vi "Deploy History.vi"() -> ()   [LabVIEW 2023]
doc: "Tools >> Systemcore >> Deploy History: lists the robot's deploys (newest first) and redeploys the one the user picks, or checks it out into the project."
panel:
  out "Status":string
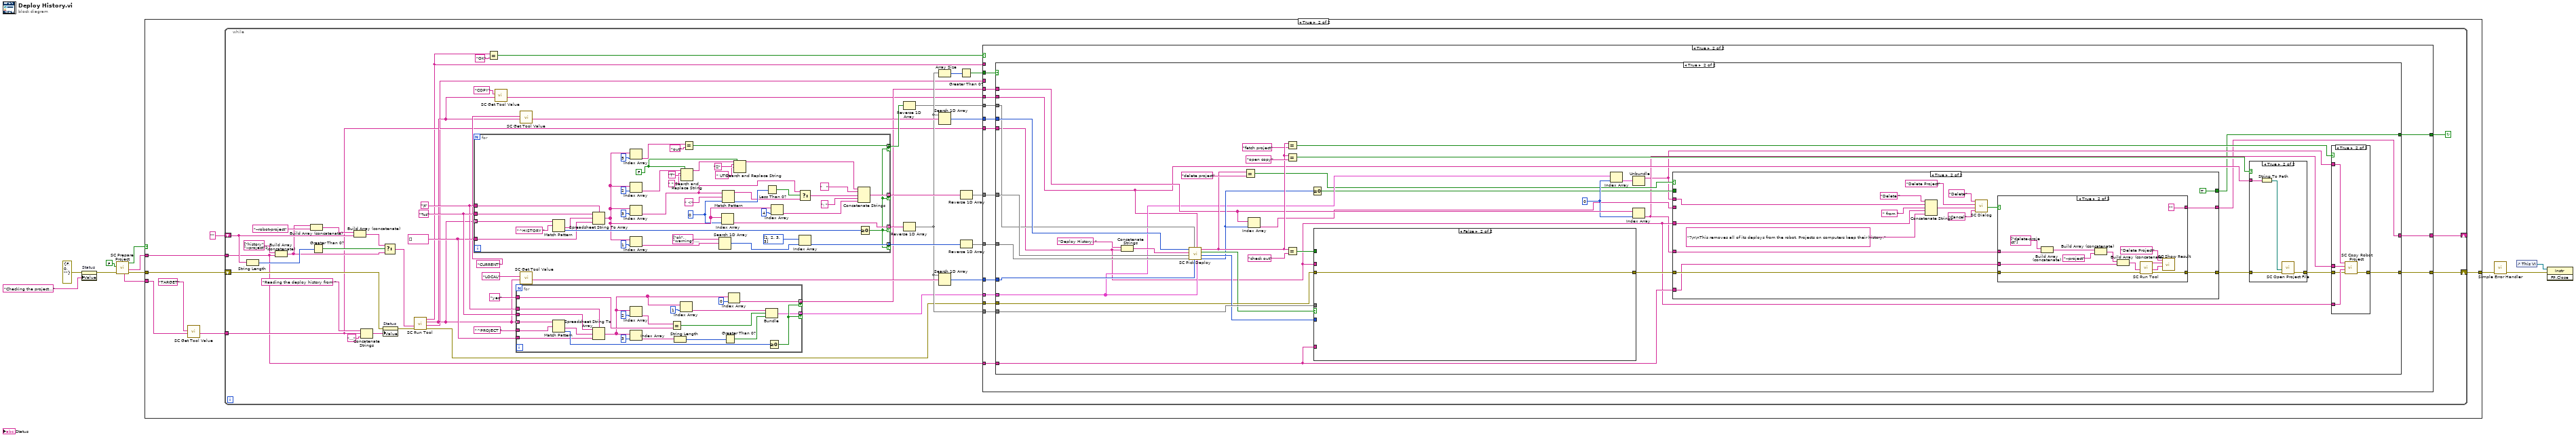
[diagram p0: block diagram]
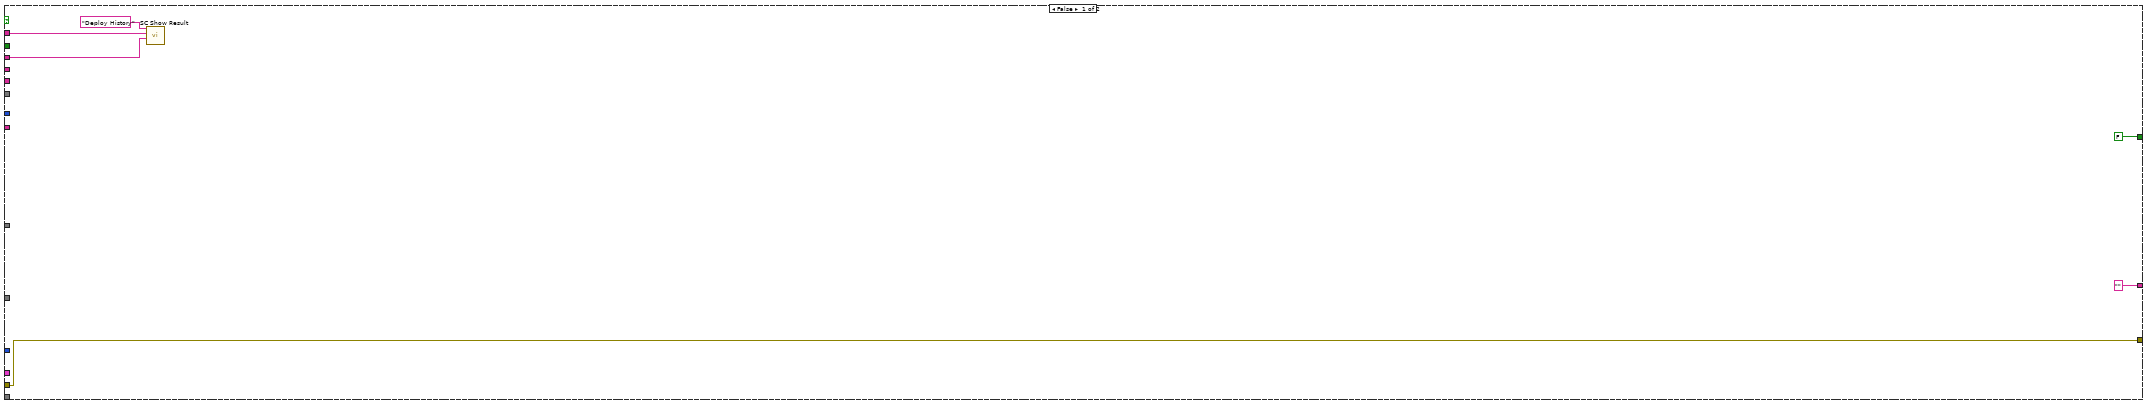
[diagram p3: hidden frame]
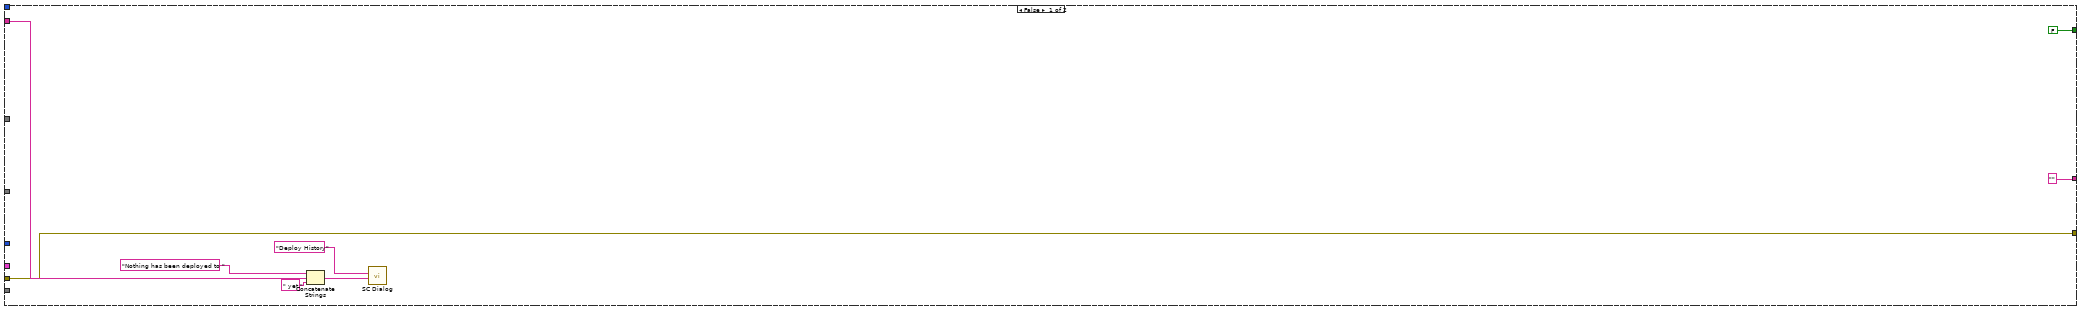
[diagram p4: hidden frame]
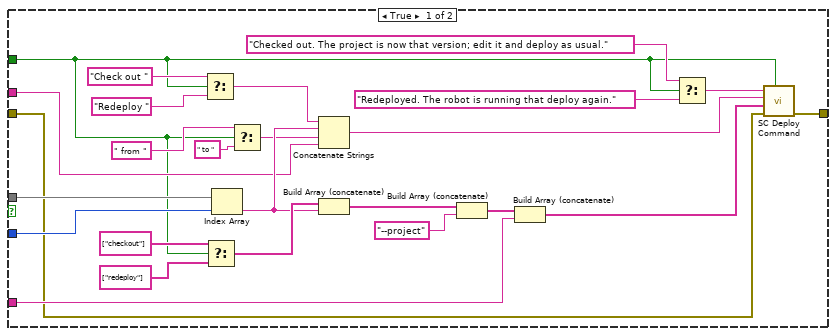
[diagram p9: hidden frame]
diagram:
  n1 = property on="Status" class="Str"(error in=errorcluster {"status"=FALSE, "code"=0, "source"=""}, "Value"="Checking the project...") -> (error out=w8:errorcluster)  [unwired: 1 in, 1 out]
  n2 = call "SC Prepare Project.vi"("error in (no error)"=w8, "save VIs?"=FALSE) -> ("error out"=w5:errorcluster, "project root"=w7:string, "ready?"=w4:bool, "tool lines"=w6:string[])  [unwired: 5 in, 1 out]
  n3 = case shown="True" w4 {
    tunnel: w7 -> [_ w17]
    tunnel: w6 -> [_ w19]
    tunnel: w5 -> [w12 w15]
    tunnel: [w12 w13] -> w3
    frame False {
    }
    frame True {
      n4 = call "SC Get Tool Value.vi"("tool lines"=w19, "key"="TARGET") -> ("value"=w16:string)  [unwired: 8 in, 1 out]
      n5 = while {
        tunnel: w17 -> [w34]
        tunnel: w16 -> [w35]
        shift-right: [w21] -> w13
        shift-left: w15 -> [w56]
        shift-right: [w22] -> _
        shift-left: "" -> [w67]
        stop <- w23 continue-if-true
        w50 = "\t"
        w51 = string[] []
        w52 = "%s"
        n6 = String Length(string=w67) -> (length=w66:i32)
        n7 = Build Array (concatenate)(string[] ["history", "--project"], w34) -> (w59:string[])
        n8 = Build Array (concatenate)(w59, "--robot-project") -> (w68:string[])
        n9 = Greater Than 0?(x=w66) -> (x > 0?=w65:bool)
        n10 = Build Array (concatenate)(w68, w67) -> (w64:string[])
        n11 = Concatenate Strings("Reading the deploy history from ", w35, "...") -> (w55:string)
        n12 = property on="Status" class="Str"(error in=w56, "Value"=w55) -> (error out=w53:errorcluster)  [unwired: 1 in, 1 out]
        n13 = Select(t=w64, s=w65, f=w59) -> (s? t:f=w54:string[])
        n14 = call "SC Run Tool.vi"("error in (no error)"=w53, "arguments"=w54) -> ("error out"=w33:errorcluster, "output"=w32:string, "tool lines"=w45:string[], "result"=w31:string)  [unwired: 4 in, 2 out]
        n15 = for {
          tunnel: w45 -> [w250] mode=indexing
          tunnel: w52 -> [w247]
          tunnel: w51 -> [w245]
          tunnel: w50 -> [w244]
          tunnel: [w213] -> w42 mode=indexing if=w210
          tunnel: [w212] -> w41 mode=indexing if=w210
          tunnel: [w211] -> w49 mode=indexing if=w210
          tunnel: [w209] -> w48 mode=indexing if=w210
          w229 = FALSE
          w227 = 0
          n16 = Match Pattern(string=w250, regular expression="^HISTORY ") -> (after substring=w246:string, offset past match=w248:i32)  [unwired: 1 in, 2 out]
          n17 = Spreadsheet String To Array(delimiter (Tab)=w244, format string=w247, spreadsheet string=w246, array type (2D Dbl)=w245) -> (array=w239:string[])
          n18 = Index Array(array=w239, index=5) -> (element=w237:string)
          n19 = Index Array(array=w239, index=2) -> (element=w235:string)
          n20 = Index Array(array=w239, index=3) -> (element=w224:string)
          n21 = Index Array(array=w239, index=1) -> (element=w216:string)
          n22 = Search and Replace String(replace all?=w229, input string=w235, search string="T", replace string=" ") -> (result string=w232:string)  [unwired: 4 in, 3 out]
          n23 = Equal?(x=w237, y="out") -> (x = y?=w209:bool)
          n24 = Search 1D Array(1D array=string[] ["ok", "warning", "broken", "error"], element=w216) -> (index of element=w214:i32)  [unwired: 1 in]
          n25 = Index Array(array=w239, index=w227) -> (element=w213:string)
          n26 = Match Pattern(string=w224, regular expression=" <", offset (0)=w227) -> (before substring=w223:string, offset past match=w226:i32)  [unwired: 2 out]
          n27 = Search and Replace String(replace all?=w229, input string=w232, search string="Z", replace string=" UTC") -> (result string=w222:string)  [unwired: 4 in, 3 out]
          n28 = Less Than 0?(x=w226) -> (x < 0?=w225:bool)
          n29 = Index Array(array=w239, index=4) -> (element=w218:string)
          n30 = Select(t=w224, s=w225, f=w223) -> (s? t:f=w220:string)
          n31 = Index Array(array=i32[] [1, 2, 3, 3], index=w214) -> (element=w211:i32)
          n32 = Concatenate Strings(w222, "   ", w220, ": ", w218) -> (w212:string)
          n33 = Greater Or Equal To 0?(x=w248) -> (x >= 0?=w210:bool)
        }
        n34 = Equal?(x=w31, y="OK") -> (x = y?=w20:bool)
        n35 = call "SC Get Tool Value.vi"("tool lines"=w45, "key"="COPY") -> ("value"=w24:string)  [unwired: 8 in, 1 out]
        n36 = for {
          tunnel: w45 -> [w272] mode=indexing
          tunnel: w52 -> [w269]
          tunnel: w51 -> [w267]
          tunnel: w50 -> [w266]
          tunnel: "^PROJECT " -> [w271]
          tunnel: "yes" -> [w261]
          tunnel: [w253] -> w26 mode=indexing if=w252
          tunnel: [w251] -> w25 mode=indexing if=w252
          n37 = Match Pattern(string=w272, regular expression=w271) -> (after substring=w268:string, offset past match=w270:i32)  [unwired: 1 in, 2 out]
          n38 = Spreadsheet String To Array(delimiter (Tab)=w266, format string=w269, spreadsheet string=w268, array type (2D Dbl)=w267) -> (array=w260:string[])
          n39 = Index Array(array=w260, index=2) -> (element=w262:string)
          n40 = Index Array(array=w260, index=3) -> (element=w258:string)
          n41 = Equal?(x=w262, y=w261) -> (x = y?=w255:bool)
          n42 = String Length(string=w258) -> (length=w257:i32)
          n43 = Index Array(array=w260, index=1) -> (element=w256:string)
          n44 = Greater Than 0?(x=w257) -> (x > 0?=w254:bool)
          n45 = Index Array(array=w260, index=0) -> (element=w253:string)
          n46 = Bundle("String"=w256, w255, w254) -> (w251:cluster{"String":string, bool, bool})  [unwired: 1 in]
          n47 = Greater Or Equal To 0?(x=w270) -> (x >= 0?=w252:bool)
        }
        n48 = call "SC Get Tool Value.vi"("tool lines"=w45, "key"="CURRENT") -> ("value"=w46:string)  [unwired: 8 in, 1 out]
        n49 = call "SC Get Tool Value.vi"("tool lines"=w45, "key"="LOCAL") -> ("value"=w43:string)  [unwired: 8 in, 1 out]
        n50 = Reverse 1D Array(array=w48) -> (reversed array=w28:bool[])
        n51 = Reverse 1D Array(array=w42) -> (reversed array=w37:string[])
        n52 = Array Size(array=w37) -> (size(s)=w40:i32)
        n53 = Search 1D Array(1D array=w37, element=w46) -> (index of element=w29:i32)  [unwired: 1 in]
        n54 = Search 1D Array(1D array=w37, element=w43) -> (index of element=w27:i32)  [unwired: 1 in]
        n55 = Greater Than 0?(x=w40) -> (x > 0?=w38:bool)
        n56 = Reverse 1D Array(array=w41) -> (reversed array=w36:string[])
        n57 = Reverse 1D Array(array=w49) -> (reversed array=w30:i32[])
        n58 = case shown="True" w20 {
          tunnel: w38 -> [_ w77]
          tunnel: w37 -> [_ w91]
          tunnel: w36 -> [_ w90]
          tunnel: w35 -> [_ w89]
          tunnel: w34 -> [_ w88]
          tunnel: w33 -> [w70 w87]
          tunnel: w32 -> [w73 _]
          tunnel: w31 -> [w72 _]
          tunnel: w30 -> [_ w86]
          tunnel: w29 -> [_ w85]
          tunnel: w28 -> [_ w84]
          tunnel: w27 -> [_ w83]
          tunnel: w26 -> [_ w82]
          tunnel: w25 -> [_ w81]
          tunnel: w24 -> [_ w80]
          tunnel: [FALSE w79] -> w23
          tunnel: ["" w78] -> w22
          tunnel: [w70 w76] -> w21
          frame False {
            n59 = call "SC Show Result.vi"("output"=w73, "result"=w72, "title"="Deploy History") -> ()  [unwired: 8 in, 1 out]
          }
          frame True {
            n60 = case shown="True" w77 {
              tunnel: w91 -> [_ w130]
              tunnel: w90 -> [_ w136]
              tunnel: w89 -> [w96 w106]
              tunnel: w88 -> [_ w112]
              tunnel: w87 -> [w92 w128]
              tunnel: w86 -> [_ w135]
              tunnel: w85 -> [_ w134]
              tunnel: w84 -> [_ w133]
              tunnel: w83 -> [_ w132]
              tunnel: w82 -> [_ w119]
              tunnel: w81 -> [_ w118]
              tunnel: w80 -> [_ w109]
              tunnel: [FALSE w101] -> w79
              tunnel: ["" w100] -> w78
              tunnel: [w92 w102] -> w76
              frame False {
                n61 = Concatenate Strings("Nothing has been deployed to ", w96, " yet.") -> (w94:string)
                n62 = call "SC Dialog.vi"("message"=w94, "window title"="Deploy History") -> ()  [unwired: 9 in, 1 out]
              }
              frame True {
                w117 = 0
                n63 = Concatenate Strings("Deploy History: ", w106) -> (w131:string)
                n64 = call "SC Pick Deploy.vi"("projects"=w118, "copy"=w109, "local"=w132, "struck"=w133, "symbols"=w135, "items"=w136, "window title"=w131, "current"=w134) -> ("project"=w120:i32, "index"=w129:i32, "chosen?"=w127:bool, "action"=w122:string)
                n65 = Equal?(x=w122, y="delete project") -> (x = y?=w111:bool)
                n66 = Index Array(array=w119, index=w120) -> (element=w113:string)
                n67 = Equal?(x=w122, y="fetch project") -> (x = y?=w103:bool)
                n68 = Equal?(x=w122, y="open copy") -> (x = y?=w108:bool)
                n69 = Equal?(x=w122, y="check out") -> (x = y?=w125:bool)
                n70 = Greater Or Equal To 0?(x=w120) -> (x >= 0?=w114:bool)
                n71 = case shown="False" w127 {
                  tunnel: w130 -> [w207 _]
                  tunnel: w129 -> [w206 _]
                  tunnel: w112 -> [w199 _]
                  tunnel: w128 -> [w184 w208]
                  tunnel: w106 -> [w191 _]
                  tunnel: w125 -> [w185 _]
                  tunnel: [w183 w208] -> w115
                  frame True {
                    n72 = Select(t="Check out ", s=w185, f="Redeploy ") -> (s? t:f=w194:string)
                    n73 = Select(t=string[] ["checkout"], s=w185, f=string[] ["redeploy"]) -> (s? t:f=w203:string[])
                    n74 = Index Array(array=w207, index=w206) -> (element=w193:string)
                    n75 = Select(t=" from ", s=w185, f=" to ") -> (s? t:f=w192:string)
                    n76 = Concatenate Strings(w194, w193, w192, w191) -> (w187:string)
                    n77 = Build Array (concatenate)(w203, w193) -> (w202:string[])
                    n78 = Build Array (concatenate)(w202, "--project") -> (w200:string[])
                    n79 = Build Array (concatenate)(w200, w199) -> (w188:string[])
                    n80 = Select(t="Checked out. The project is now that version; edit it and deploy as usual.", s=w185, f="Redeployed. The robot is running that deploy again.") -> (s? t:f=w186:string)
                    n81 = call "SC Deploy Command.vi"("close project first?"=w185, "error in (no error)"=w184, "arguments"=w188, "title"=w187, "OK message"=w186) -> ("error out"=w183:errorcluster)  [unwired: 5 in, 1 out]
                  }
                  frame False {
                  }
                }
                n82 = Index Array(array=w118, index=w117) -> (element=w116:cluster{"String":string, bool, bool})
                n83 = Unbundle(w116) -> ("String"=w104:string)  [unwired: 2 out]
                n84 = Index Array(array=w119, index=w117) -> (element=w105:string)
                n85 = case shown="True" w111 {
                  tunnel: w115 -> [w151 w158]
                  tunnel: w114 -> [w150 _]
                  tunnel: w113 -> [w149 _]
                  tunnel: w105 -> [_ w157]
                  tunnel: w104 -> [_ w166]
                  tunnel: w106 -> [_ w164]
                  tunnel: w112 -> [_ w156]
                  tunnel: [w151 w154] -> w110
                  tunnel: [w150 TRUE] -> w101
                  tunnel: [w149 w152] -> w100
                  frame False {
                  }
                  frame True {
                    n86 = Concatenate Strings("Delete ", w166, " from ", w164, "?\n\nThis removes all of its deploys from the robot. Projects on computers keep their history.") -> (w162:string)
                    n87 = call "SC Dialog.vi"("Cancel text"="Cancel", "message"=w162, "window title"="Delete Project", "OK text"="Delete") -> ("OK?"=w155:bool)  [unwired: 7 in]
                    n88 = case shown="True" w155 {
                      tunnel: w158 -> [w169 w175]
                      tunnel: w157 -> [w168 w181]
                      tunnel: w156 -> [_ w177]
                      tunnel: [w169 w171] -> w154
                      tunnel: [w168 ""] -> w152
                      frame False {
                      }
                      frame True {
                        n89 = Build Array (concatenate)(string[] ["delete-project"], w181) -> (w180:string[])
                        n90 = Build Array (concatenate)(w180, "--project") -> (w178:string[])
                        n91 = Build Array (concatenate)(w178, w177) -> (w176:string[])
                        n92 = call "SC Run Tool.vi"("error in (no error)"=w175, "arguments"=w176) -> ("error out"=w171:errorcluster, "output"=w174:string, "result"=w173:string)  [unwired: 4 in, 3 out]
                        n93 = call "SC Show Result.vi"("output"=w174, "result"=w173, "title"="Delete Project") -> ()  [unwired: 8 in, 1 out]
                      }
                    }
                  }
                }
                n94 = case shown="True" w108 {
                  tunnel: w110 -> [w144 w146]
                  tunnel: w109 -> [_ w148]
                  tunnel: [w144 w145] -> w107
                  frame False {
                  }
                  frame True {
                    n95 = String To Path(string=w148) -> (path=w147:path)
                    n96 = call "SC Open Project File.vi"("error in (no error)"=w146, "path"=w147) -> ("error out"=w145:errorcluster)  [unwired: 9 in]
                  }
                }
                n97 = case shown="True" w103 {
                  tunnel: w107 -> [w138 w140]
                  tunnel: w106 -> [_ w143]
                  tunnel: w105 -> [_ w142]
                  tunnel: w104 -> [_ w141]
                  tunnel: [w138 w139] -> w102
                  frame False {
                  }
                  frame True {
                    n98 = call "SC Copy Robot Project.vi"("error in (no error)"=w140, "target"=w143, "root"=w142, "name"=w141) -> ("error out"=w139:errorcluster)  [unwired: 6 in, 1 out]
                  }
                }
              }
            }
          }
        }
      }
    }
  }
  n99 = call <vilib>:"Simple Error Handler.vi"("error in (no error)"=w3) -> ("error out"=w1:errorcluster)  [unwired: 4 in, 4 out]
  n100 = control-ref of="This VI"() -> (w2:refnum<vi>)
  n101 = invoke class="Instr" method="FP.Close"(reference=w2, error in=w1) -> ()  [unwired: 1 in, 3 out]
